vi "hand_dataset_generation_v001.vi"() -> ()   [LabVIEW 2025]
uses:
  <vilib>/MakerHub/Leap/Private/Type Defs/Frame.ctl
  <vilib>/MakerHub/Leap/Private/Type Defs/Gesture Key Tap.ctl
  <vilib>/MakerHub/Leap/Private/Type Defs/Gesture Common.ctl
  <vilib>/MakerHub/Leap/Private/Type Defs/Gesture Type.ctl
  <vilib>/MakerHub/Leap/Private/Type Defs/Gesture State.ctl
  <vilib>/MakerHub/Leap/Private/Type Defs/Vector.ctl
  <vilib>/MakerHub/Leap/Private/Type Defs/Gesture Circle.ctl
  <vilib>/MakerHub/Leap/Private/Type Defs/Gesture Screen Tap.ctl
  <vilib>/MakerHub/Leap/Private/Type Defs/Gesture Swipe.ctl
  <vilib>/MakerHub/Leap/Private/Type Defs/Hand.ctl
  <vilib>/MakerHub/Leap/Private/Type Defs/Pointable.ctl
  <vilib>/MakerHub/Leap/Private/Type Defs/Pointable Type.ctl
  <vilib>/MakerHub/Leap/Private/Type Defs/Pointable Zone.ctl
  <vilib>/MakerHub/Leap/LMH-Leap.lvlib
panel:
  in  "Namefile":string="Hand_"
  in  "Save?":bool
  in  "Class":dbl
  out "Fingers XYZ":dbl[](array[numeric])
  out "Palm XYZ":dbl[](array[numeric])
  out "Frame":T1
  in  "stop":bool
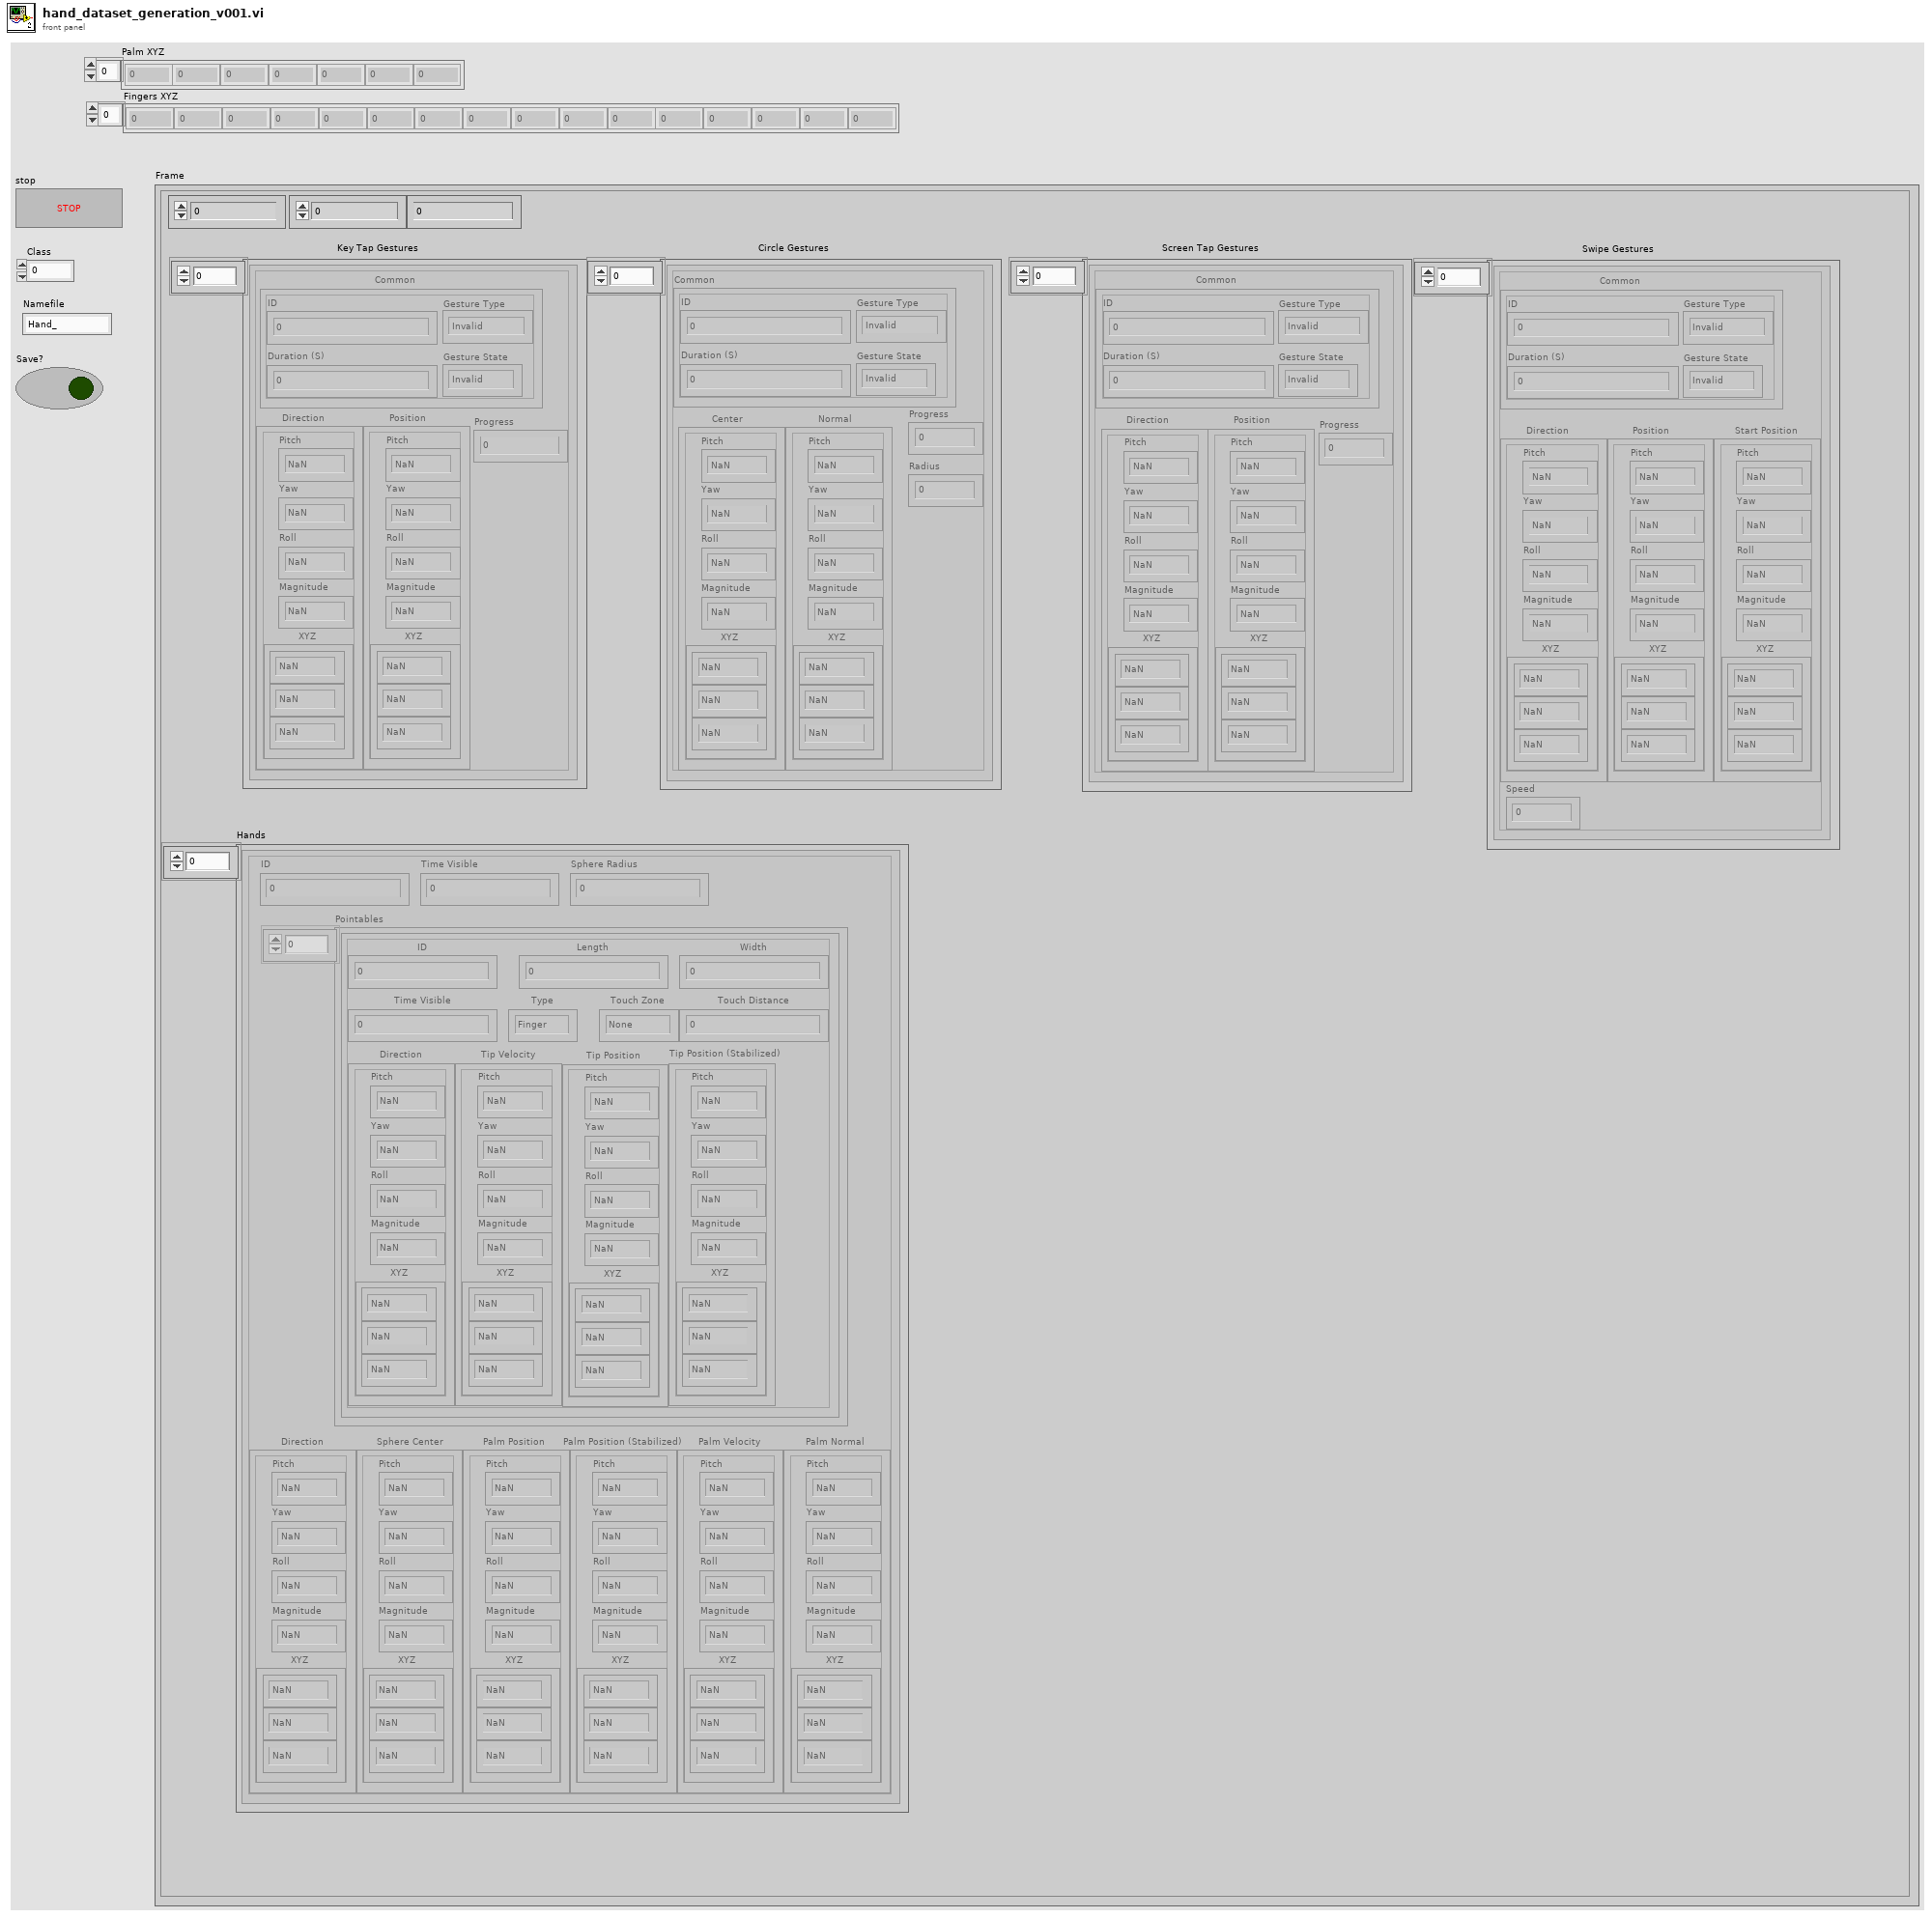
[diagram p1: front panel]
types:
  T1 = typedef "LMH-Leap.lvlib/Frame.ctl" = cluster{"ID":i64, "Timestamp":i64, "Current FPS":dbl, "Key Tap Gestures":T2[], "Circle Gestures":T7[], "Screen Tap Gestures":T8[], "Swipe Gestures":T9[], "Hands":T10[]}
  T2 = typedef "LMH-Leap.lvlib/Gesture Key Tap.ctl" = cluster{"Common":T3, "Direction":T6, "Position":T6, "Progress":dbl}
  T3 = typedef "LMH-Leap.lvlib/Gesture Common.ctl" = cluster{"ID":dbl, "Duration (S)":dbl, "Gesture Type":T4, "Gesture State":T5}
  T4 = typedef "LMH-Leap.lvlib/Gesture Type.ctl" = enum16{"Invalid", "Swipe", "Circle", "Screen Tap", "Key Tap"}
  T5 = typedef "LMH-Leap.lvlib/Gesture State.ctl" = enum16{"Invalid", "Start", "Update", "Stop"}
  T6 = typedef "LMH-Leap.lvlib/Vector.ctl" = cluster{"Pitch":sgl, "Yaw":sgl, "Roll":sgl, "Magnitude":sgl, "XYZ":sgl[]}
  T7 = typedef "LMH-Leap.lvlib/Gesture Circle.ctl" = cluster{"Common":T3, "Center":T6, "Normal":T6, "Progress":dbl, "Radius":dbl}
  T8 = typedef "LMH-Leap.lvlib/Gesture Screen Tap.ctl" = cluster{"Common":T3, "Direction":T6, "Position":T6, "Progress":dbl}
  T9 = typedef "LMH-Leap.lvlib/Gesture Swipe.ctl" = cluster{"Common":T3, "Direction":T6, "Position":T6, "Start Position":T6, "Speed":dbl}
  T10 = typedef "LMH-Leap.lvlib/Hand.ctl" = cluster{"Palm Normal":T6, "Palm Position":T6, "Palm Velocity":T6, "Direction":T6, "Palm Position (Stabilized)":T6, "Sphere Center":T6, "Pointables":T11[], "ID":i32, "Time Visible":sgl, "Sphere Radius":sgl}
  T11 = typedef "LMH-Leap.lvlib/Pointable.ctl" = cluster{"Type":T12, "Touch Zone":T13, "ID":i32, "Length":dbl, "Width":dbl, "Time Visible":dbl, "Touch Distance":dbl, "Direction":T6, "Tip Position":T6, "Tip Velocity":T6, "Tip Position (Stabilized)":T6}
  T12 = typedef "LMH-Leap.lvlib/Pointable Type.ctl" = enum16{"Finger", "Tool"}
  T13 = typedef "LMH-Leap.lvlib/Pointable Zone.ctl" = enum16{"None", "Hovering", "Touching"}
  T14 = enum16{"open", "replace", "create", "open or create", "replace or create", "replace or create with confirmation"}
  T15 = typedef "LMH-Leap.lvlib/Leap Handle.ctl" = cluster{"LeapCSharp":refnum<k24>}
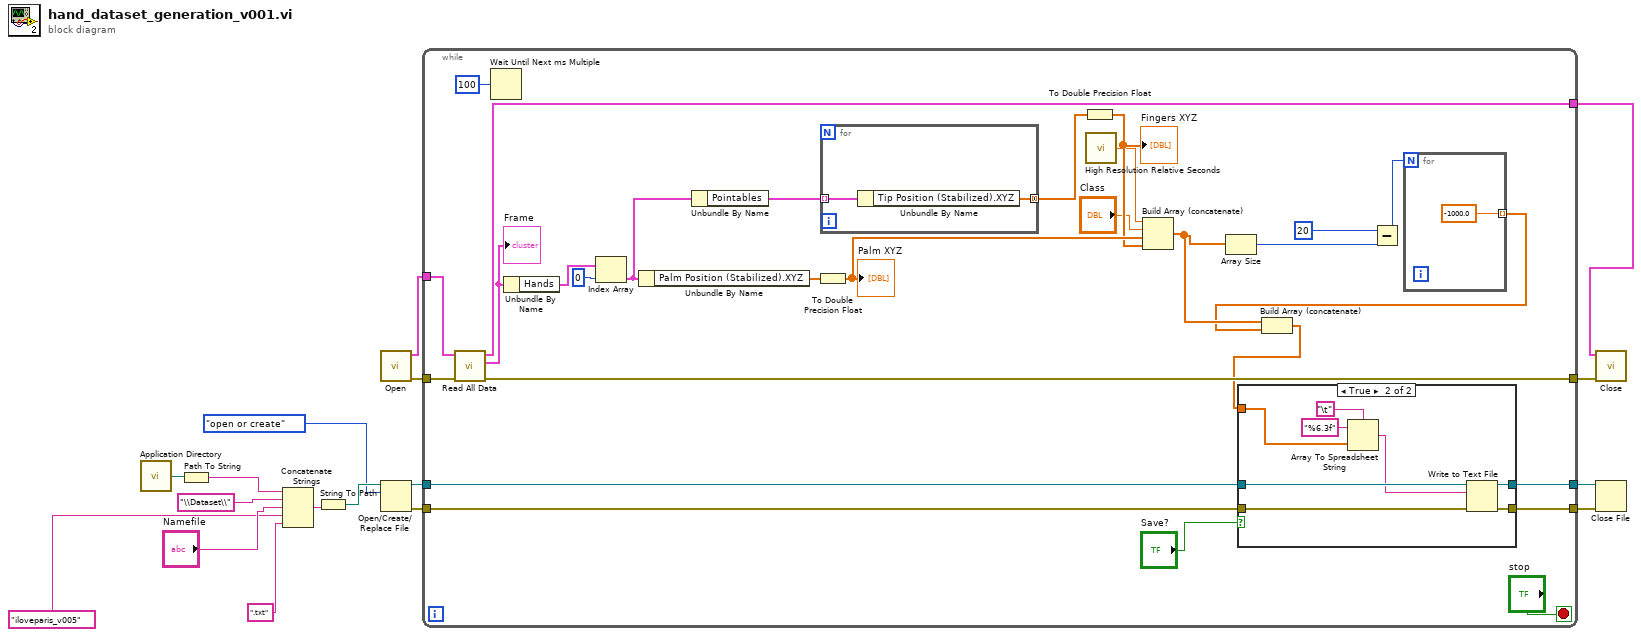
[diagram p0: block diagram]
diagram:
  n1 = call <vilib>:"Application Directory.vi"() -> ("Application Directory"=w9:path)
  n2 = Path To String(path=w9) -> (string=w8:string)
  n3 = Concatenate Strings(w8, "\\Dataset\\" ("string"), "Namefile", "iloveparis_v005" ("time format string (%c)"), ".txt" ("string")) -> (w6:string)
  n4 = String To Path(string=w6) -> (path=w5:path)
  n5 = call <vilib>:"Open.vi"() -> ("Error Out"=w16:errorcluster, "Leap Handle"=w17:T15)  [unwired: 10 in]
  n6 = Open/Create/Replace File(file path (use dialog)=w5, operation (0:open)=T14."open or create") -> (refnum out=w12:refnum<file>, error out=w13:errorcluster)  [unwired: 4 in, 1 out]
  n7 = while {
    tunnel: w17 -> [w45]
    tunnel: w16 -> [w44]
    tunnel: [w43] -> w15
    tunnel: [w42] -> w14
    tunnel: w13 -> [w27]
    tunnel: w12 -> [w24]
    tunnel: [w26] -> w11
    tunnel: [w25] -> w10
    stop <- "stop" stop-if-true
    n8 = call <vilib>:"Read All Data.vi"("Error In"=w44, "Leap Handle"=w45) -> ("Error Out"=w42:errorcluster, "Frame"=w39:T1, "Leap Handle"=w43:T15)  [unwired: 6 in, 1 out]
    "Frame" <- w39
    n9 = Wait Until Next ms Multiple(millisecond multiple=u32 100) -> ()  [unwired: 1 out]
    n10 = Unbundle By Name(w39) -> ("Hands"=w38:T10[])
    n11 = Index Array(array=w38, index=0) -> (element=w36:T10)
    n12 = Unbundle By Name(w36) -> ("Palm Position (Stabilized).XYZ"=w35:sgl[])
    n13 = Unbundle By Name(w36) -> ("Pointables"=w31:T11[])
    n14 = To Double Precision Float(number=w35) -> (double precision float=w33:dbl[])
    "Palm XYZ" <- w33
    n15 = for {
      tunnel: w31 -> [w58] mode=indexing
      tunnel: [w57] -> w34 mode=concatenating
      n16 = Unbundle By Name(w58) -> ("Tip Position (Stabilized).XYZ"=w57:sgl[])
    }
    n17 = To Double Precision Float(number=w34) -> (double precision float=w32:dbl[])
    "Fingers XYZ" <- w32
    n18 = call <vilib>:"High Resolution Relative Seconds.vi"() -> ("relative seconds"=w30:dbl)
    n19 = Build Array (concatenate)(w30, "Class", w33, w32) -> (w20:dbl[])
    n20 = Array Size(array=w20) -> (size(s)=w23:i32)
    n21 = Subtract(x=20, y=w23) -> (x-y=w21:i32)
    n22 = for {
      N: w21 -> [_]
      tunnel: [-1000.0] -> w19 mode=indexing
    }
    n23 = Build Array (concatenate)(w20, w19) -> (w18:dbl[])
    n24 = case shown="True" "Save?" {
      tunnel: w27 -> [w48 w56]
      tunnel: [w48 w55] -> w26
      tunnel: [w47 w54] -> w25
      tunnel: w18 -> [_ w52]
      tunnel: w24 -> [w47 w53]
      frame False {
      }
      frame True {
        n25 = Array To Spreadsheet String(delimiter (Tab)="\t", array=w52, 3:"%6.3f" ("format string")) -> (spreadsheet string=w50:string)
        n26 = Write to Text File(file (use dialog)=w53, text=w50, error in=w56) -> (refnum out=w54:refnum<file>, error out=w55:errorcluster)  [unwired: 1 in, 1 out]
      }
    }
  }
  n27 = call <vilib>:"Close.vi"("Error In"=w14, "Leap Handle"=w15) -> ()  [unwired: 9 in, 1 out]
  n28 = Close File(refnum=w10, error in=w11) -> ()  [unwired: 2 out]
